vi "SLSC Read Properties.vi"(5 "Read Only?":bool, 7 "Default Only?":bool, 8 "error in (no error)":errorcluster, 9 "Popup?":bool, 10 "SLSC Device":refnum<k21>, 11 "SLSC EDS module in":T1) -> (0 "error out":errorcluster, 3 "SLSC EDS module out":T1)   [LabVIEW 2020, in "SLSC EDS API.lvlib"]
uses:
  SLSC EDS API.lvlib
  JSON parsing/EDSjsonStructure.ctl
  JSON parsing/enum.ctl
  JSON parsing/property.ctl
  JSON parsing/command.ctl
  JSON parsing/scale.ctl
  JSON parsing/physicalChannel.ctl
  JSON parsing/register.ctl
  <vilib>/SLSC/Initialize Session with Devices.vi
  <vilib>/SLSC/Get Generic Property (Bool).vi
  <vilib>/SLSC/Get Generic Property (String).vi
  <vilib>/SLSC/Get Generic Property (DBL).vi
  <vilib>/SLSC/Get Generic Property (I32).vi
  <vilib>/SLSC/Get Generic Property (I64).vi
  <vilib>/SLSC/Get Generic Property (U32).vi
  <vilib>/SLSC/Get Generic Property (U64).vi
  <vilib>/SLSC/Close Session.vi
  <vilib>/SLSC/SLSC.lvlib
  SLSC CD API/SLSC CD System Explorer/SLSC CD System Explorer.lvlib
  SLSC CD API/SLSC CD Shared/SLSC CD Shared.lvlib
panel:
  # "not working\nregisterMap->registers->initialValue"
  # "not working\nregisterMap->registers->initialValue"
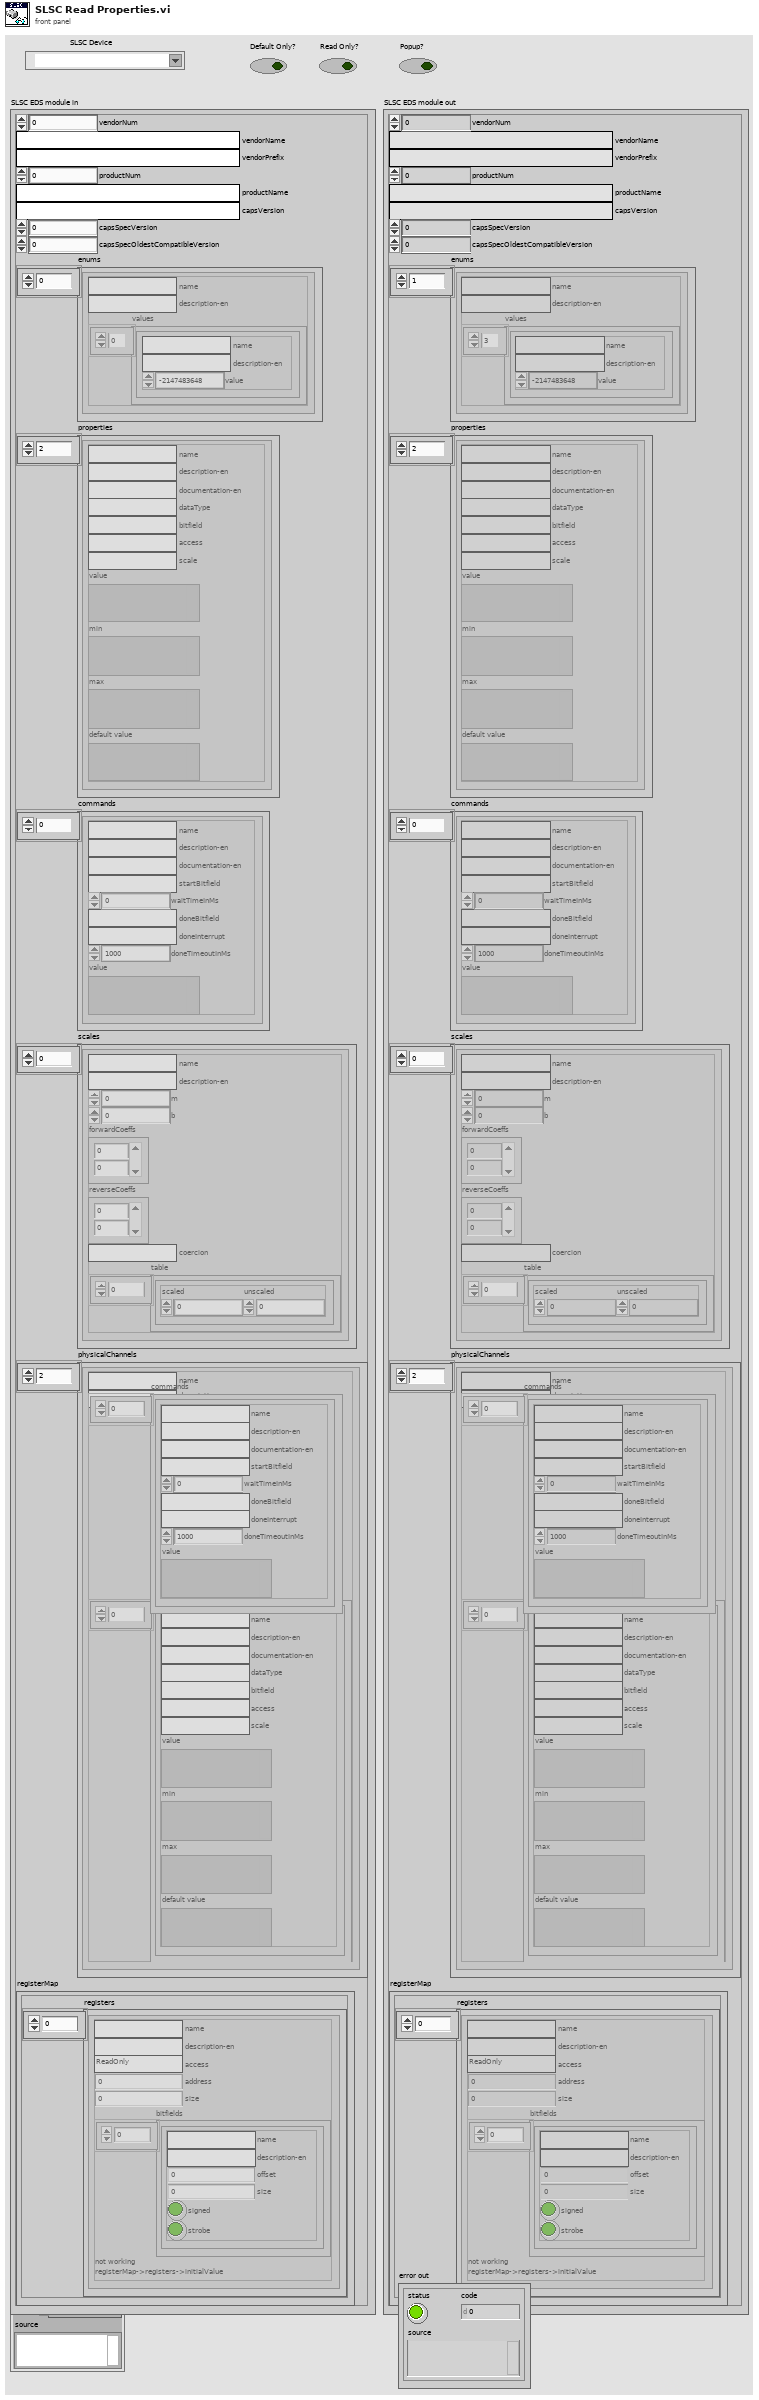
[diagram p1: front panel]
types:
  T1 = typedef "EDSjsonStructure.ctl" = cluster{"vendorNum":u32, "vendorName":string, "vendorPrefix":string, "productNum":u32, "productName":string, "capsVersion":string, "capsSpecVersion":u32, "capsSpecOldestCompatibleVersion":u32, "enums":T2[], "properties":T3[], "commands":T4[], "scales":T5[], "physicalChannels":T6[], "registerMap":cluster{"registers":T7[]}}
  T2 = typedef "enum.ctl" = cluster{"name":string, "description-en":string, "values":cluster{"name":string, "description-en":string, "value":i32}[]}
  T3 = typedef "property.ctl" = cluster{"name":string, "description-en":string, "documentation-en":string, "dataType":string, "bitfield":string, "access":string, "scale":string, "value":variant, "min":variant, "max":variant, "default value":variant}
  T4 = typedef "command.ctl" = cluster{"name":string, "description-en":string, "documentation-en":string, "startBitfield":string, "waitTimeInMs":i32, "doneBitfield":string, "doneInterrupt":string, "doneTimeoutInMs":i32, "value":variant}
  T5 = typedef "scale.ctl" = cluster{"name":string, "description-en":string, "m":dbl, "b":dbl, "forwardCoeffs":dbl[], "reverseCoeffs":dbl[], "coercion":string, "table":cluster{"scaled":dbl, "unscaled":dbl}[]}
  T6 = typedef "physicalChannel.ctl" = cluster{"name":string, "description-en":string, "commands":T4[], "properties":T3[]}
  T7 = typedef "register.ctl" = cluster{"name":string, "description-en":string, "access":string, "address":u32, "size":u32, "bitfields":cluster{"name":string, "description-en":string, "offset":u32, "size":u32, "signed":bool, "strobe":bool}[]}
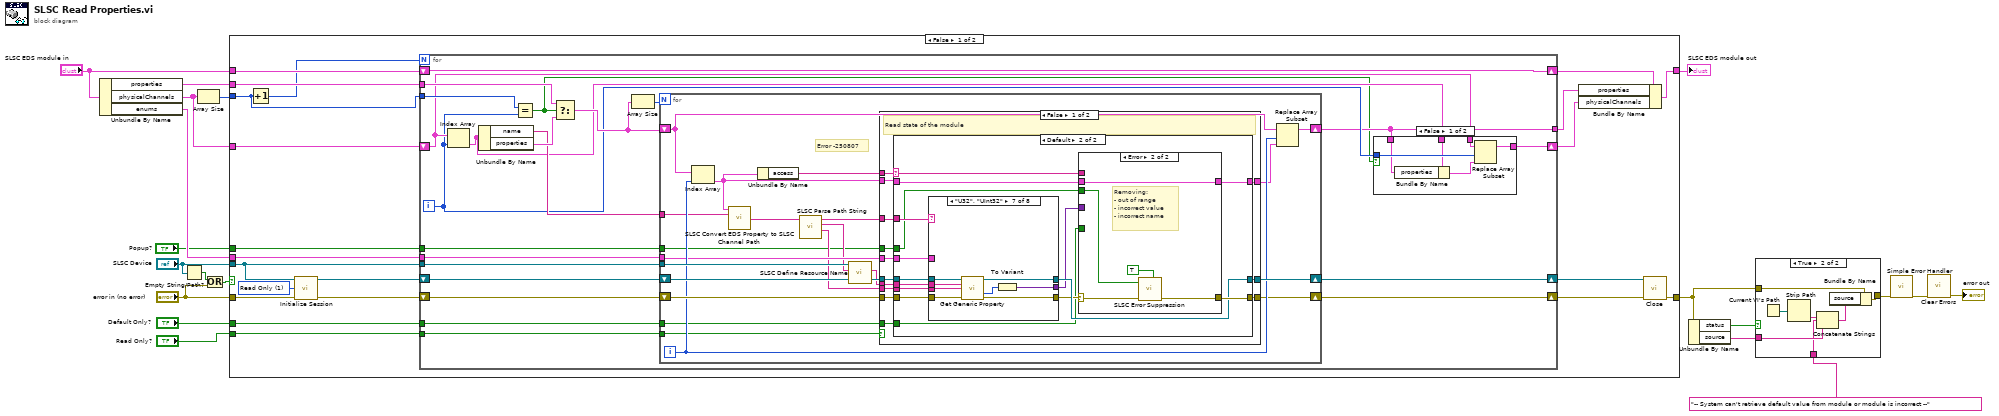
[diagram p0: block diagram]
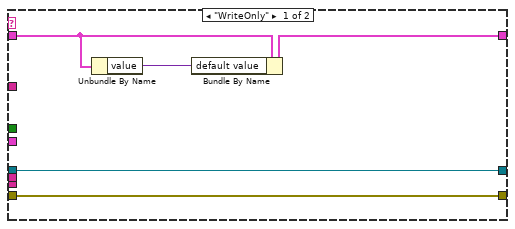
[diagram p4: hidden frame]
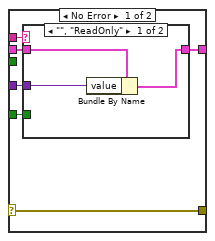
[diagram p5: hidden frame]
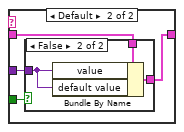
[diagram p6: hidden frame]
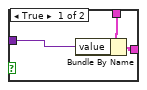
[diagram p7: hidden frame]
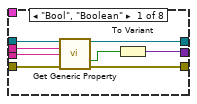
[diagram p8: hidden frame]
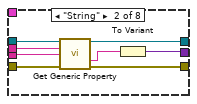
[diagram p9: hidden frame]
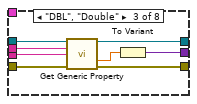
[diagram p10: hidden frame]
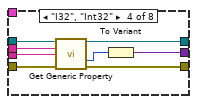
[diagram p11: hidden frame]
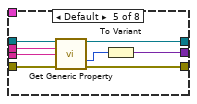
[diagram p12: hidden frame]
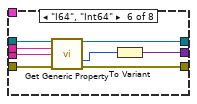
[diagram p13: hidden frame]
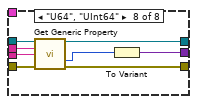
[diagram p14: hidden frame]
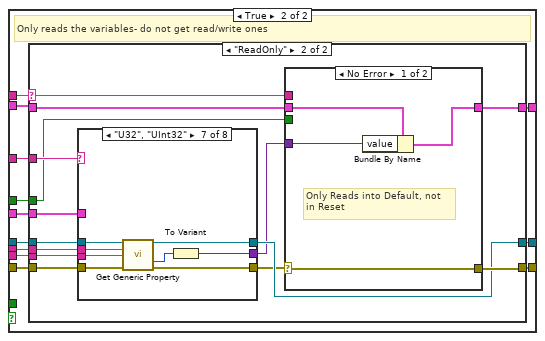
[diagram p15: hidden frame]
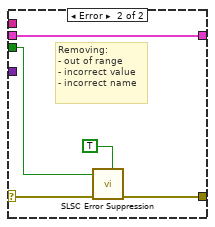
[diagram p17: hidden frame]
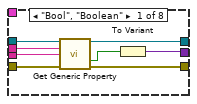
[diagram p18: hidden frame]
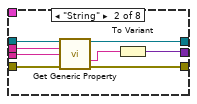
[diagram p19: hidden frame]
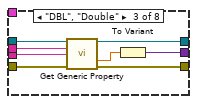
[diagram p20: hidden frame]
diagram:
  n1 = Unbundle By Name("SLSC EDS module in") -> ("properties"=w4:T3[], "physicalChannels"=w5:T6[], "enums"=w7:T2[])
  n2 = Empty String/Path?(string/path="SLSC Device") -> (empty?=w9:bool)
  n3 = Array Size(array=w5) -> (size(s)=w6:i32)
  n4 = Or(x=w9, y="error in (no error)") -> (x .or. y?=w12:bool)
  n5 = case shown="False" w12 {
    tunnel: "SLSC EDS module in" -> [w41 w316]
    tunnel: [w27 w316] -> w20
    tunnel: "SLSC Device" -> [w36 _]
    tunnel: [w38 w315] -> w17
    tunnel: "error in (no error)" -> [w34 w315]
    tunnel: w7 -> [w33 _]
    tunnel: w6 -> [w29 _]
    tunnel: w5 -> [w32 _]
    tunnel: w4 -> [w31 _]
    tunnel: "Read Only?" -> [w23 _]
    tunnel: "Default Only?" -> [w22 _]
    tunnel: "Popup?" -> [w21 _]
    frame False {
      w24 = 1 items=["None"=0, "Read Only"=1, "Read/Write"=3] ("reservation access (Read/Write)")
      n6 = Increment(x=w29) -> (x+1=w30:i32)
      n7 = call-poly <vilib>:"Initialize Session.vi"("devices"=w36, "reservation access (Read/Write)"=w24, "error in (no error)"=w34) -> ("session out"=w37:refnum<k21>, "error out"=w35:errorcluster)  [unwired: 11 in]
      n8 = for {
        N: w30 -> [_]
        tunnel: w36 -> [w59]
        shift-right: [w52] -> w28
        shift-left: w41 -> [w52]
        shift-right: [w63] -> w40
        shift-left: w37 -> [w60]
        shift-right: [w62] -> w39
        shift-left: w35 -> [w58]
        tunnel: w33 -> [w57]
        tunnel: w31 -> [w56]
        tunnel: [w47] -> w26
        tunnel: w29 -> [w51]
        shift-right: [w46] -> w25
        shift-left: w32 -> [w50]
        tunnel: w23 -> [w44]
        tunnel: w22 -> [w43]
        tunnel: w21 -> [w42]
        i -> [w49]
        n9 = Index Array(array=w50, index=w49) -> (element=w48:T6)
        n10 = Unbundle By Name(w48) -> ("name"=w53:string, "properties"=w54:T3[])
        n11 = Equal?(x=w51, y=w49) -> (x = y?=w45:bool)
        n12 = Select(t=w56, s=w45, f=w54) -> (s? t:f=w55:T3[])
        n13 = Array Size(array=w55) -> (size(s)=w61:i32)
        n14 = for {
          N: w61 -> [_]
          shift-right: [w90] -> w47
          shift-left: w55 -> [w91]
          shift-right: [w88] -> w63
          shift-left: w60 -> [w85]
          tunnel: w59 -> [w83]
          tunnel: w53 -> [w76]
          tunnel: w57 -> [w77]
          shift-right: [w78] -> w62
          shift-left: w58 -> [w87]
          tunnel: w44 -> [w73]
          tunnel: w43 -> [w72]
          tunnel: w42 -> [w71]
          i -> [w82]
          # "Error -250807"
          n15 = Index Array(array=w91, index=w82) -> (element=w80:T3)
          n16 = call "SLSC Convert EDS Property to SLSC Channel Path.vi"("property"=w80, "Physical Channel"=w76) -> ("SLSC Channel Path"=w86:string)  [unwired: 7 in, 6 out]
          n17 = Unbundle By Name(w80) -> ("access"=w81:string)
          n18 = call "SLSC Parse Path String.vi"("SLSC Channel Path"=w86) -> ("Property or Command"=w74:string, "Physical Channel"=w75:string, "Datatype"=w89:string)  [unwired: 7 in, 1 out]
          n19 = call "SLSC Define Resource Name.vi"("SLSC Item"=w75, "SLSC Module Name"=w83) -> ("Resource"=w84:string)  [unwired: 9 in]
          n20 = case shown="False" w73 {
            tunnel: w89 -> [w104 w224]
            tunnel: [w103 w223] -> w88
            tunnel: w87 -> [w102 w222]
            tunnel: w85 -> [w101 w221]
            tunnel: w84 -> [w100 w220]
            tunnel: w81 -> [w99 w219]
            tunnel: w80 -> [w98 w218]
            tunnel: [w97 w217] -> w79
            tunnel: [w96 w216] -> w78
            tunnel: w77 -> [w95 w215]
            tunnel: w74 -> [w94 w214]
            tunnel: w72 -> [w93 _]
            tunnel: w71 -> [w92 w213]
            frame False {
              # "Read state of the module"
              n21 = case shown="Default" w99 {
                selector: w99 -> [_ w114]
                tunnel: w104 -> [_ w115]
                tunnel: [w109 w116] -> w103
                tunnel: w102 -> [w108 w124]
                tunnel: [w108 w117] -> w96
                tunnel: w94 -> [_ w123]
                tunnel: w101 -> [w109 w122]
                tunnel: w100 -> [_ w121]
                tunnel: w98 -> [w106 w120]
                tunnel: [w107 w119] -> w97
                tunnel: w95 -> [_ w118]
                tunnel: w93 -> [_ w111]
                tunnel: w92 -> [_ w110]
                frame "WriteOnly" {
                  n22 = Unbundle By Name(w106) -> ("value"=w105:variant)
                  n23 = Bundle By Name(cluster=w106, "default value"=w105) -> (w107:T3)
                }
                frame Default {
                  n24 = case shown="\"U32\", \"UInt32\"" w115 {
                    tunnel: w122 -> [w156 w164 w172 w180 w188 w196 w204 w212]
                    tunnel: [w155 w163 w171 w179 w187 w195 w203 w211] -> w116
                    tunnel: w123 -> [w154 w162 w170 w178 w186 w194 w202 w210]
                    tunnel: w124 -> [w153 w161 w169 w177 w185 w193 w201 w209]
                    tunnel: [w152 w160 w168 w176 w184 w192 w200 w208] -> w112
                    tunnel: [w149 w157 w165 w175 w183 w191 w199 w205] -> w113
                    tunnel: w121 -> [w151 w159 w166 w173 w181 w189 w197 w207]
                    tunnel: w118 -> [_ _ _ _ _ _ _ _]
                    frame "Bool", "Boolean" {
                      n25 = call-poly <vilib>:"Get Generic Property.vi"("session in"=w156, "resources"=w151, "property"=w154, "error in (no error)"=w153) -> ("session out"=w155:refnum<k21>, "property value"=w150:bool, "error out"=w152:errorcluster)  [unwired: 9 in]
                      n26 = To Variant(anything=w150) -> (Variant=w149:variant)
                    }
                    frame "String" {
                      n27 = call-poly <vilib>:"Get Generic Property.vi"("session in"=w164, "resources"=w159, "property"=w162, "error in (no error)"=w161) -> ("session out"=w163:refnum<k21>, "property value"=w158:string, "error out"=w160:errorcluster)  [unwired: 9 in]
                      n28 = To Variant(anything=w158) -> (Variant=w157:variant)
                    }
                    frame "DBL", "Double" {
                      n29 = call-poly <vilib>:"Get Generic Property.vi"("session in"=w172, "resources"=w166, "property"=w170, "error in (no error)"=w169) -> ("session out"=w171:refnum<k21>, "property value"=w167:dbl, "error out"=w168:errorcluster)  [unwired: 9 in]
                      n30 = To Variant(anything=w167) -> (Variant=w165:variant)
                    }
                    frame "I32", "Int32" {
                      n31 = call-poly <vilib>:"Get Generic Property.vi"("session in"=w180, "resources"=w173, "property"=w178, "error in (no error)"=w177) -> ("session out"=w179:refnum<k21>, "property value"=w174:i32, "error out"=w176:errorcluster)  [unwired: 9 in]
                      n32 = To Variant(anything=w174) -> (Variant=w175:variant)
                    }
                    frame Default {
                      n33 = call-poly <vilib>:"Get Generic Property.vi"("session in"=w188, "resources"=w181, "property"=w186, "error in (no error)"=w185) -> ("session out"=w187:refnum<k21>, "property value"=w182:i32, "error out"=w184:errorcluster)  [unwired: 9 in]
                      n34 = To Variant(anything=w182) -> (Variant=w183:variant)
                    }
                    frame "I64", "Int64" {
                      n35 = call-poly <vilib>:"Get Generic Property.vi"("session in"=w196, "resources"=w189, "property"=w194, "error in (no error)"=w193) -> ("session out"=w195:refnum<k21>, "property value"=w190:i64, "error out"=w192:errorcluster)  [unwired: 9 in]
                      n36 = To Variant(anything=w190) -> (Variant=w191:variant)
                    }
                    frame "U32", "UInt32" {
                      n37 = call-poly <vilib>:"Get Generic Property.vi"("session in"=w204, "resources"=w197, "property"=w202, "error in (no error)"=w201) -> ("session out"=w203:refnum<k21>, "property value"=w198:u32, "error out"=w200:errorcluster)  [unwired: 9 in]
                      n38 = To Variant(anything=w198) -> (Variant=w199:variant)
                    }
                    frame "U64", "UInt64" {
                      n39 = call-poly <vilib>:"Get Generic Property.vi"("session in"=w212, "resources"=w207, "property"=w210, "error in (no error)"=w209) -> ("session out"=w211:refnum<k21>, "property value"=w206:u64, "error out"=w208:errorcluster)  [unwired: 9 in]
                      n40 = To Variant(anything=w206) -> (Variant=w205:variant)
                    }
                  }
                  n41 = case shown="Error" w112 {
                    selector: w112 -> [w128 w147]
                    tunnel: w120 -> [w130 w148]
                    tunnel: [w129 w148] -> w119
                    tunnel: w113 -> [w127 _]
                    tunnel: [w128 w146] -> w117
                    tunnel: w114 -> [w126 _]
                    tunnel: w111 -> [w125 _]
                    tunnel: w110 -> [_ w144]
                    frame No Error {
                      n42 = case shown="\"\", \"ReadOnly\"" w126 {
                        tunnel: w130 -> [w133 w137]
                        tunnel: [w132 w136] -> w129
                        tunnel: w127 -> [w131 w135]
                        tunnel: w125 -> [_ w134]
                        frame "", "ReadOnly" {
                          n43 = Bundle By Name(cluster=w133, "value"=w131) -> (w132:T3)
                        }
                        frame Default {
                          n44 = case shown="False" w134 {
                            tunnel: w137 -> [w140 w143]
                            tunnel: [w139 w142] -> w136
                            tunnel: w135 -> [w138 w141]
                            frame True {
                              n45 = Bundle By Name(cluster=w140, "value"=w138) -> (w139:T3)
                            }
                            frame False {
                              n46 = Bundle By Name(cluster=w143, "value"=w141, "default value"=w141) -> (w142:T3)
                            }
                          }
                        }
                      }
                    }
                    frame Error {
                      # "Removing: \n- out of range\n- incorrect value\n- incorrect name"
                      n47 = call "SLSC Error Suppression.vi"("error in (no error)"=w147, "Popup Error?"=w144, "Clear All Error?"=TRUE) -> ("error out"=w146:errorcluster)  [unwired: 6 in, 1 out]
                    }
                  }
                }
              }
            }
            frame True {
              # "Only reads the variables- do not get read/write ones"
              n48 = case shown="\"ReadOnly\"" w219 {
                selector: w219 -> [_ w231]
                tunnel: w224 -> [_ w232]
                tunnel: [w227 w233] -> w223
                tunnel: w222 -> [w226 w241]
                tunnel: [w226 w234] -> w216
                tunnel: w214 -> [_ w240]
                tunnel: w221 -> [w227 w239]
                tunnel: w220 -> [_ w238]
                tunnel: w218 -> [w225 w237]
                tunnel: [w225 w236] -> w217
                tunnel: w215 -> [_ w235]
                tunnel: w213 -> [_ w228]
                frame "ReadWrite", "WriteOnly", Default {
                }
                frame "ReadOnly" {
                  n49 = case shown="\"U32\", \"UInt32\"" w232 {
                    tunnel: w239 -> [w258 w266 w274 w282 w290 w298 w306 w314]
                    tunnel: [w257 w265 w273 w281 w289 w297 w305 w313] -> w233
                    tunnel: w240 -> [w256 w264 w272 w280 w288 w296 w304 w312]
                    tunnel: w241 -> [w255 w263 w271 w279 w287 w295 w303 w311]
                    tunnel: [w254 w262 w270 w278 w286 w294 w302 w310] -> w229
                    tunnel: [w251 w259 w267 w277 w285 w293 w301 w307] -> w230
                    tunnel: w238 -> [w253 w261 w268 w275 w283 w291 w299 w309]
                    tunnel: w235 -> [_ _ _ _ _ _ _ _]
                    frame "Bool", "Boolean" {
                      n50 = call-poly <vilib>:"Get Generic Property.vi"("session in"=w258, "resources"=w253, "property"=w256, "error in (no error)"=w255) -> ("session out"=w257:refnum<k21>, "property value"=w252:bool, "error out"=w254:errorcluster)  [unwired: 9 in]
                      n51 = To Variant(anything=w252) -> (Variant=w251:variant)
                    }
                    frame "String" {
                      n52 = call-poly <vilib>:"Get Generic Property.vi"("session in"=w266, "resources"=w261, "property"=w264, "error in (no error)"=w263) -> ("session out"=w265:refnum<k21>, "property value"=w260:string, "error out"=w262:errorcluster)  [unwired: 9 in]
                      n53 = To Variant(anything=w260) -> (Variant=w259:variant)
                    }
                    frame "DBL", "Double" {
                      n54 = call-poly <vilib>:"Get Generic Property.vi"("session in"=w274, "resources"=w268, "property"=w272, "error in (no error)"=w271) -> ("session out"=w273:refnum<k21>, "property value"=w269:dbl, "error out"=w270:errorcluster)  [unwired: 9 in]
                      n55 = To Variant(anything=w269) -> (Variant=w267:variant)
                    }
                    frame "I32", "Int32" {
                      n56 = call-poly <vilib>:"Get Generic Property.vi"("session in"=w282, "resources"=w275, "property"=w280, "error in (no error)"=w279) -> ("session out"=w281:refnum<k21>, "property value"=w276:i32, "error out"=w278:errorcluster)  [unwired: 9 in]
                      n57 = To Variant(anything=w276) -> (Variant=w277:variant)
                    }
                    frame Default {
                      n58 = call-poly <vilib>:"Get Generic Property.vi"("session in"=w290, "resources"=w283, "property"=w288, "error in (no error)"=w287) -> ("session out"=w289:refnum<k21>, "property value"=w284:i32, "error out"=w286:errorcluster)  [unwired: 9 in]
                      n59 = To Variant(anything=w284) -> (Variant=w285:variant)
                    }
                    frame "I64", "Int64" {
                      n60 = call-poly <vilib>:"Get Generic Property.vi"("session in"=w298, "resources"=w291, "property"=w296, "error in (no error)"=w295) -> ("session out"=w297:refnum<k21>, "property value"=w292:i64, "error out"=w294:errorcluster)  [unwired: 9 in]
                      n61 = To Variant(anything=w292) -> (Variant=w293:variant)
                    }
                    frame "U32", "UInt32" {
                      n62 = call-poly <vilib>:"Get Generic Property.vi"("session in"=w306, "resources"=w299, "property"=w304, "error in (no error)"=w303) -> ("session out"=w305:refnum<k21>, "property value"=w300:u32, "error out"=w302:errorcluster)  [unwired: 9 in]
                      n63 = To Variant(anything=w300) -> (Variant=w301:variant)
                    }
                    frame "U64", "UInt64" {
                      n64 = call-poly <vilib>:"Get Generic Property.vi"("session in"=w314, "resources"=w309, "property"=w312, "error in (no error)"=w311) -> ("session out"=w313:refnum<k21>, "property value"=w308:u64, "error out"=w310:errorcluster)  [unwired: 9 in]
                      n65 = To Variant(anything=w308) -> (Variant=w307:variant)
                    }
                  }
                  n66 = case shown="No Error" w229 {
                    selector: w229 -> [w243 w249]
                    tunnel: w237 -> [w245 w250]
                    tunnel: [w244 w250] -> w236
                    tunnel: w230 -> [w242 _]
                    tunnel: [w243 w248] -> w234
                    tunnel: w231 -> [_ _]
                    tunnel: w228 -> [_ w246]
                    frame No Error {
                      # "Only Reads into Default, not\nin Reset"
                      n67 = Bundle By Name(cluster=w245, "value"=w242) -> (w244:T3)
                    }
                    frame Error {
                      # "Removing: \n- out of range\n- incorrect value\n- incorrect name"
                      n68 = call "SLSC Error Suppression.vi"("error in (no error)"=w249, "Popup Error?"=w246, "Clear All Error?"=TRUE) -> ("error out"=w248:errorcluster)  [unwired: 6 in, 1 out]
                    }
                  }
                }
              }
            }
          }
          n69 = Replace Array Subset(array=w91, new element=w79, index=w82) -> (w90:T3[])
        }
        n70 = case shown="False" w45 {
          tunnel: w50 -> [w69 w70]
          tunnel: w49 -> [w68 _]
          tunnel: w48 -> [w67 _]
          tunnel: w47 -> [w66 _]
          tunnel: [w64 w70] -> w46
          frame False {
            n71 = Bundle By Name(cluster=w67, "properties"=w66) -> (w65:T6)
            n72 = Replace Array Subset(array=w69, new element=w65, index=w68) -> (w64:T6[])
          }
          frame True {
          }
        }
      }
      n73 = Bundle By Name(cluster=w28, "properties"=w26, "physicalChannels"=w25) -> (w27:T1)
      n74 = call-poly <vilib>:"Close.vi"("session in"=w40, "error in (no error)"=w39) -> ("error out"=w38:errorcluster)  [unwired: 13 in]
    }
    frame True {
    }
  }
  "SLSC EDS module out" <- w20
  n75 = Unbundle By Name(w17) -> ("status"=w14:bool, "source"=w15:string)
  n76 = case shown="True" w14 {
    tunnel: w17 -> [w317 w324]
    tunnel: [w317 w323] -> w16
    tunnel: w15 -> [_ w322]
    tunnel: "-- System can't retrieve default value from module or module is incorrect --" -> [_ w320]
    frame False {
    }
    frame True {
      n77 = Current VI's Path() -> (path=w319:path)
      n78 = Strip Path(path=w319) -> (name=w318:string)  [unwired: 1 out]
      n79 = Concatenate Strings(w318, w320, w322) -> (w321:string)
      n80 = Bundle By Name(cluster=w324, "source"=w321) -> (w323:errorcluster)
    }
  }
  n81 = call <vilib>:"Simple Error Handler.vi"("error in (no error)"=w16) -> ("error out"=w19:errorcluster)  [unwired: 4 in, 4 out]
  n82 = call <vilib>:"Clear Errors.vi"("error in (no error)"=w19) -> ("error out"=→"error out":errorcluster)  [unwired: 5 in, 1 out]
